vi "Stop Core.vi"(10 "final error code":i32, 11 "Nested in":refnum<class "ChannelManagerUI.lvclass">) -> (3 "Nested out":refnum<class "ChannelManagerUI.lvclass">)   [LabVIEW 2021, in "Channel.lvlib" / "ChannelManagerUI.lvlib" / "ChannelManagerUI.lvclass"]
doc: "(<B>Filename</B>: Actor Framework.lvlib:Actor.lvclass:Stop Core.vi)\n\nDefines what the actor does before it stops. Use the <B>final error code</B> input to determine whether the actor shut down in response to an error.\n\nBy default, this method does nothing. A descendant class may override it to define behavior, such as shutting down any processes the actor initiated in its override of the Actor Core method."
uses:
  ChannelManagerUI.lvclass
  <vilib>/event_ctls.llb/usereventprio.ctl
  ChannelManagerUI.lvclass/ChannelManagerUI.ctl
  ChannelsManager/ChannelsManager/ChannelsManager.lvclass
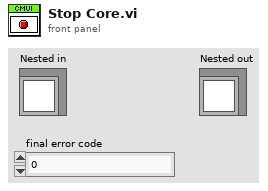
[diagram p1: front panel]
types:
  T1 = typedef "usereventprio.ctl" = enum32{"high priority", "normal priority"}
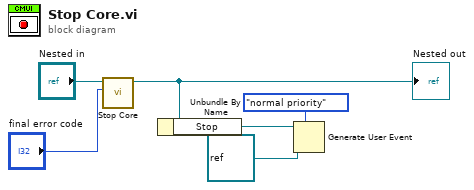
[diagram p0: block diagram]
diagram:
  n1 = call-parent "Stop Core.vi"("final error code"="final error code", "Actor in"="Nested in") -> ("Actor out"=w4:refnum<class "ChannelManagerUI.lvclass">)  [unwired: 9 in]
  "Nested out" <- w4
  n2 = Unbundle By Name(w4) -> ("Stop"=w3:refnum<user-event>)
  n3 = Generate User Event(priority (normal)=usereventprio."normal priority", user event=w3, event data cluster=refnum<class> refnum ("event data")) -> ()  [unwired: 1 in, 2 out]
